vi "init data cluster.vi"(0 "data clusters in":T2[](array[typedef]), 5 "shared memory name":string, 7 "channel classification":T3, 9 "data type":T1, 11 "error in":errorcluster, 12 "index":i32[](array[numeric])) -> (4 "data clusters out":T2[](array[typedef]), 6 "sequential tags?":bool, 15 "error out":errorcluster)   [LabVIEW 2014, in "Shared Memory runtime.lvclass"]
uses:
  Shared Memory runtime.lvclass
  <vilib>/NI/Tag Bus Module Framework/channel/channel classification.ctl
  channel runtime.ctl
  <vilib>/NI/Tag Bus/tag/Data Type.ctl
  <vilib>/NI/NI Linux RT IPC/Shared Memory/Controls/reference.ctl
  <vilib>/NI/NI Linux RT IPC/Shared Memory/Classes/Shared Memory/Shared Memory.lvclass
  <vilib>/NI/NI Linux RT IPC/Shared Memory/Controls/file mode.ctl
  <vilib>/NI/NI Linux RT IPC/Shared Memory/Linux RT IPC.Shared Memory.lvlib
  <vilib>/NI/Tag Bus/tag/tag descriptor.lvclass
  <vilib>/NI/Tag Bus Module Framework/channel/TBM channel.lvclass
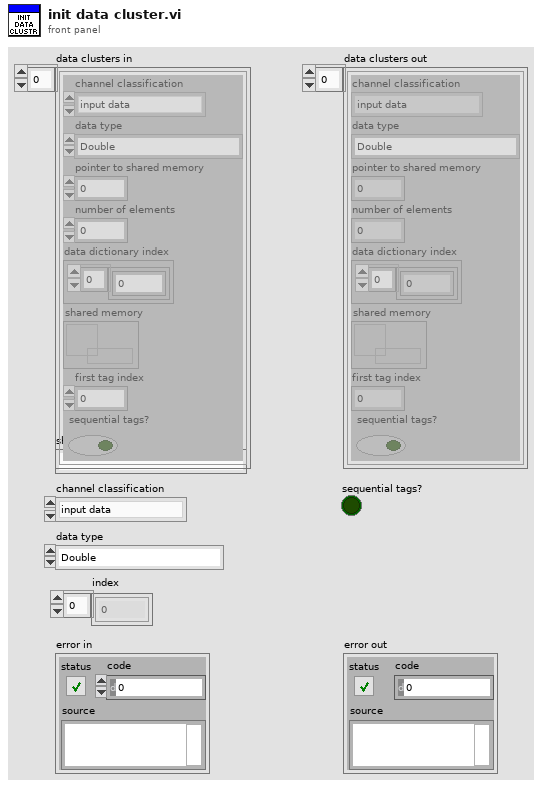
[diagram p1: front panel]
types:
  T1 = typedef "tag bus.lvlib/tag descriptor.lvclass/Data Type.ctl" = enum16{"Double", "Single", "I64", "I32", "I16", "I8", "U64", "U32", "U16", "U8", "Boolean", "String", "Array of Double", "Array of Single", "Array of I64", "Array of I32", "Array of I16", "Array of I8", "Array of U64", "Array of U32", "Array of U16", "Array of U8", "Array of Boolean", "Array of String"}
  T2 = typedef "Shared Memory runtime.lvclass/channel runtime.ctl" = cluster{"channel classification":T3, "data type":T1, "pointer to shared memory":u64, "number of elements":u64, "data dictionary index":cluster{i32[]}, "shared memory":T4, "first tag index":i32, "sequential tags?":bool}
  T3 = typedef "TBM channel.lvclass/channel classification.ctl" = enum16{"input data", "output data", "processing parameter", "processing result"}
  T4 = typedef "Linux RT IPC.Shared Memory.lvlib/reference.ctl" = refnum<data-value>
  T5 = cluster{"owner":cluster{"read":bool, "write":bool, "execute":bool}, "group":cluster{"read":bool, "write":bool, "execute":bool}, "everyone":cluster{"read":bool, "write":bool, "execute":bool}}
  T6 = typedef "Linux RT IPC.Shared Memory.lvlib/file mode.ctl" = enum16{"open", "create/replace"}
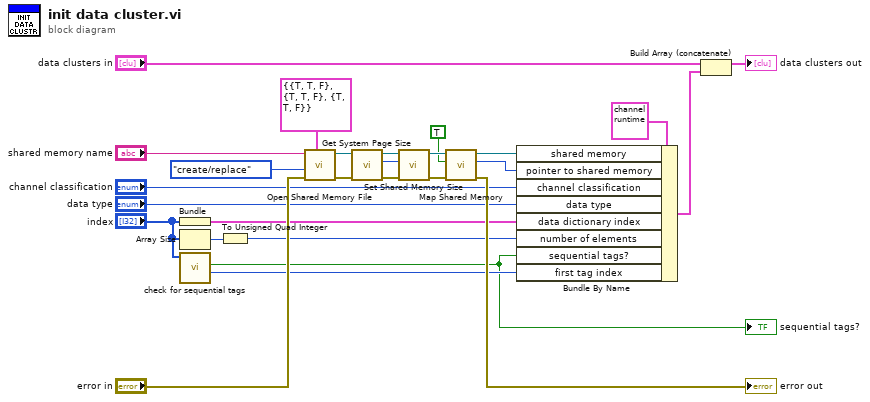
[diagram p0: block diagram]
diagram:
  n1 = Bundle("index"="index") -> (w23:cluster{"index":i32[]})  [unwired: 1 in]
  n2 = Array Size(array="index") -> (size(s)=w7:i32)
  n3 = call "check for sequential tags.vi"("indices in"="index") -> ("first index"=w3:i32, "sequential?"=w2:bool)  [unwired: 8 in, 1 out]
  "sequential tags?" <- w2
  n4 = To Unsigned Quad Integer(1:w7) -> (0:w6:u64)
  n5 = call <vilib>:"Open Shared Memory File.vi"("permissions (0664)"=T5 {"owner"={"read"=TRUE, "write"=TRUE, "execute"=FALSE}, "group"={"read"=TRUE, "write"=TRUE, "execute"=FALSE}, "everyone"={"read"=TRUE, "write"=TRUE, "execute"=FALSE}}, "error in (no error)"="error in", "file mode (open)"=file_mode."create/replace" ("file mode (default: open)"), "shared memory name"="shared memory name") -> ("error out"=w18:errorcluster, "shared memory out"=w14:T4)  [unwired: 6 in]
  n6 = call <vilib>:"Get System Page Size.vi"("error in (no error)"=w18, "shared memory in"=w14) -> ("error out"=w19:errorcluster, "page size (bytes)"=w17:u32, "shared memory out"=w15:T4)  [unwired: 7 in]
  n7 = call <vilib>:"Set Shared Memory Size.vi"("error in (no error)"=w19, "size (bytes)"=w17, "shared memory in"=w15) -> ("error out"=w20:errorcluster, "shared memory out"=w16:T4)  [unwired: 7 in]
  n8 = call <vilib>:"Map Shared Memory.vi"("error in (no error)"=w20, "close file descriptor on success? (F)"=TRUE, "shared memory in"=w16) -> ("error out"=→"error out":errorcluster, "pointer to shared memory"=w22:u64, "shared memory out"=w25:T4)  [unwired: 6 in]
  n9 = Bundle By Name(cluster=T2 {"channel classification"=enum."input data", "data type"=enum."Double", "pointer to shared memory"=0, "number of elements"=0, "data dictionary index"={[]}, "shared memory"=refnum, "first tag index"=0, "sequential tags?"=FALSE} ("runtime"), "shared memory"=w25, "pointer to shared memory"=w22, "channel classification"="channel classification", "data type"="data type", "data dictionary index"=w23, "number of elements"=w6, "sequential tags?"=w2, "first tag index"=w3) -> (w4:T2)
  n10 = Build Array (concatenate)("data clusters in", w4) -> (→"data clusters out":T2[])
